vi "Lithography Data to Overlay.vi"(8 "error in":errorcluster, 10 "Lithography Data":T2(array[cluster]), 11 "BigMAQ in":refnum<class "BigMAQ.lvclass">) -> (0 "error out":errorcluster, 2 "Disabled Overlays":string[](array[string]), 3 "BigMAQ out":refnum<class "BigMAQ.lvclass">)   [LabVIEW 2019, in "BigMAQ.lvclass"]
uses:
  BigMAQ.lvclass
  <userlib>/LevyLab/Relay Box/Typedefs/Resistor--enum.ctl
  BigMAQ.lvclass/BigMAQ.ctl
  Overlay.ctl
  <vilib>/LabVIEW Open Source Project/Cryptographic Functions/MD5/MD5.vi
  <vilib>/LabVIEW Open Source Project/Cryptographic Functions/MD5/MD5.lvclass
  <vilib>/LabVIEW Open Source Project/Cryptographic Functions/MD5/MD5.lvlib
  <userlib>/LevyLab/Relay Box/Relay-Box.lvclass
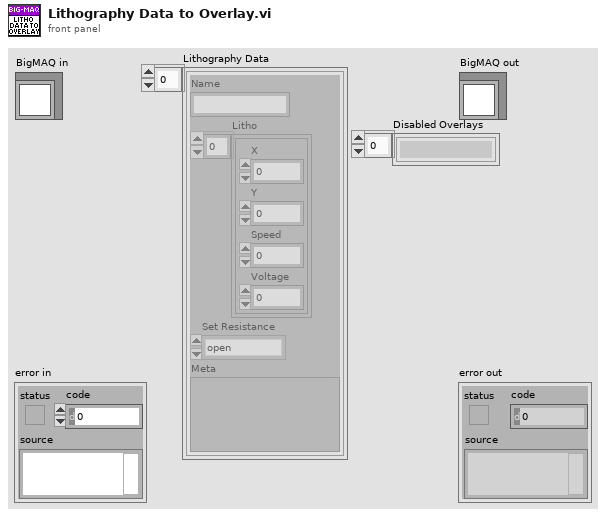
[diagram p1: front panel]
types:
  T1 = typedef "Relay-Box.lvclass/Resistor--enum.ctl" = enum16{"open", "discharge tip", "0 ohms", "100k ohm", "10M ohm", "1G ohm"}
  T2 = cluster{"Name":string, "Litho":cluster{"X":dbl, "Y":dbl, "Speed":dbl, "Voltage":dbl}[], "Set Resistance":T1, "Meta":variant}[]
  T3 = typedef "BigMAQ.lvclass/Overlay.ctl" = cluster{"Name":string, "Data":cluster{"Points":cluster{"X":dbl, "Y":dbl}[], "Voltages":dbl[]}, "Changes":cluster{"MD5 Digest":string, "Changed?":bool}}
  T4 = cluster{"X":dbl, "Y":dbl, "Speed":dbl, "Voltage":dbl}[]
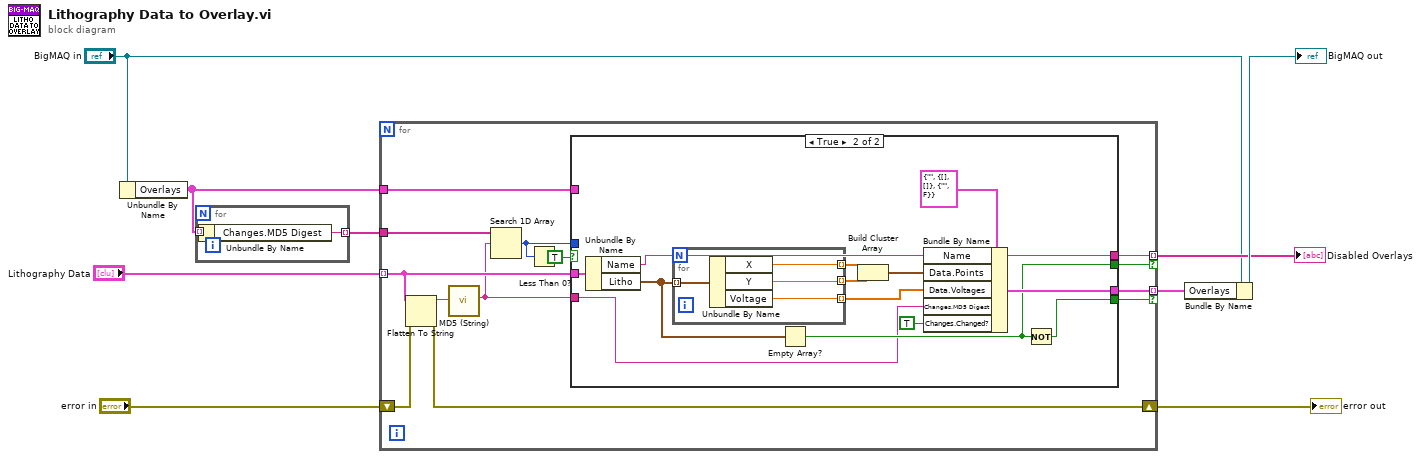
[diagram p0: block diagram]
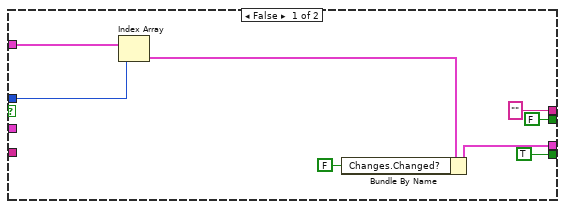
[diagram p2: hidden frame]
diagram:
  n1 = Unbundle By Name("BigMAQ in") -> ("Overlays"=w4:T3[])
  n2 = for {
    tunnel: w4 -> [w11] mode=indexing
    tunnel: [w10] -> w3 mode=indexing
    n3 = Unbundle By Name(w11) -> ("Changes.MD5 Digest"=w10:string)
  }
  n4 = for {
    tunnel: "Lithography Data" -> [w20] mode=indexing
    tunnel: [w24] -> w9 mode=indexing if=w21
    tunnel: [w23] -> w6 mode=indexing if=w22
    tunnel: w4 -> [w17]
    tunnel: w3 -> [w19]
    shift-right: [w15] -> w1
    shift-left: "error in" -> [w16]
    n5 = Flatten To String(anything=w20, error in (no error)=w16) -> (data string=w14:string, error out=w15:errorcluster)  [unwired: 2 in, 1 out]
    n6 = call <vilib>:"MD5 (String).vi"("message"=w14) -> ("MD5 hash"=w13:string)  [unwired: 10 in]
    n7 = Search 1D Array(1D array=w19, element=w13) -> (index of element=w18:i32)  [unwired: 1 in]
    n8 = Less Than 0?(x=w18) -> ()  [unwired: 1 out]
    n9 = case shown="True" TRUE {
      tunnel: [w27 w39] -> w24
      tunnel: ["" ("Name") w38] -> w23
      tunnel: [FALSE ("empty?") w37] -> w22
      tunnel: [TRUE w36] -> w21
      tunnel: w20 -> [_ w35]
      tunnel: w18 -> [w31 _]
      tunnel: w17 -> [w32 _]
      tunnel: w13 -> [_ w34]
      frame False {
        n10 = Index Array(array=w32, index=w31) -> (element=w25:T3)
        n11 = Bundle By Name(cluster=w25, "Changes.Changed?"=FALSE) -> (w27:T3)
      }
      frame True {
        n12 = Unbundle By Name(w35) -> ("Name"=w38:string, "Litho"=w44:T4)
        n13 = for {
          tunnel: w44 -> [w46] mode=indexing
          tunnel: [w49] -> w43 mode=indexing
          tunnel: [w48] -> w41 mode=indexing
          tunnel: [w47] -> w42 mode=indexing
          n14 = Unbundle By Name(w46) -> ("X"=w48:dbl, "Y"=w47:dbl, "Voltage"=w49:dbl)
        }
        n15 = Empty Array?(array=w44) -> (empty?=w37:bool)
        n16 = Build Cluster Array(w41, w42) -> (w40:cluster{"X":dbl, "Y":dbl}[])
        n17 = Bundle By Name(cluster=T3 {"Name"="", "Data"={"Points"=[], "Voltages"=[]}, "Changes"={"MD5 Digest"="", "Changed?"=FALSE}} ("Overlay"), "Name"=w38, "Data.Points"=w40, "Data.Voltages"=w43, "Changes.MD5 Digest"=w34, "Changes.Changed?"=TRUE) -> (w39:T3)
        n18 = Not(x=w37) -> (.not. x?=w36:bool)
      }
    }
  }
  "error out" <- w1
  "Disabled Overlays" <- w6
  n19 = Bundle By Name(cluster="BigMAQ in", "Overlays"=w9) -> (→"BigMAQ out":refnum<class "BigMAQ.lvclass">)
